vi "VIH Utility - UI - Set Key Focus to a Control.vi"(8 "error in":errorcluster, 11 "Ctl Refnum":refnum<vi>) -> (0 "error out":errorcluster, 2 "Key Focus out":bool)   [LabVIEW 2014]
doc: "::: VI Helpeks :::\nCopyright (c) 2000-2026 Konstantin Shifershteyn. All rights reserved."
panel:
  out "Attempt":i32
  # "VI Helpeks\nCopyright (c) 2012-2026 Konstantin Shifershteyn"
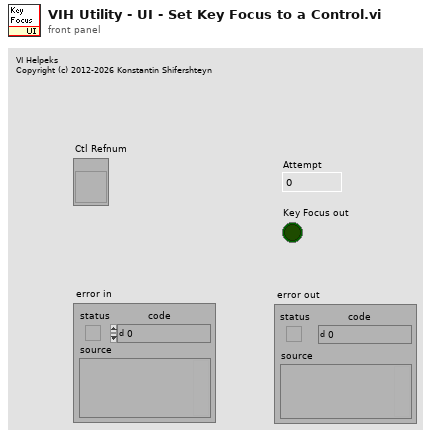
[diagram p1: front panel]
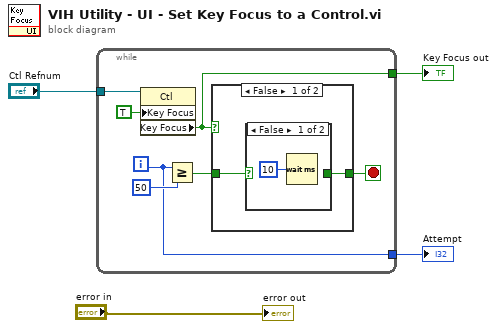
[diagram p0: block diagram]
diagram:
  n1 = while {
    tunnel: "Ctl Refnum" -> [w11]
    tunnel: [w6] -> w2
    tunnel: [w5] -> w1
    i -> [w6]
    stop <- w7 stop-if-true
    n2 = property class="Ctl"(reference=w11, "Key Focus"=TRUE) -> ("Key Focus"=w5:bool)  [unwired: 1 in, 2 out]
    n3 = Greater Or Equal?(x=w6, y=50) -> (x >= y?=w8:bool)
    n4 = case shown="False" w5 {
      selector: w5 -> [_ w16]
      tunnel: w8 -> [w13 _]
      tunnel: [w12 w16] -> w7
      frame False {
        n5 = case shown="False" w13 {
          selector: w13 -> [_ w15]
          tunnel: [_ w15] -> w12
          frame False {
            n6 = Wait (ms)(milliseconds to wait=u32 10) -> ()  [unwired: 1 out]
          }
          frame True {
          }
        }
      }
      frame True {
      }
    }
  }
  "Attempt" <- w2
  "Key Focus out" <- w1
  "error out" <- "error in"
